vi "Read Device - Protocol.vi"(8 "error in (no error)":errorcluster, 11 "LTE in":refnum<class "LTE.lvclass">) -> (0 "error out":errorcluster, 2 "Device - Protocol":T1, 3 "LTE out":refnum<class "LTE.lvclass">)   [LabVIEW 2023, in "ANRITSU Call Box.lvlib" / "LTE.lvclass"]
uses:
  LTE.lvclass
  LTE.lvclass/LTE.ctl
  Type Definition/Call Device - Protocol Type Selector.ctl
  ANRITSU Call Box.lvlib
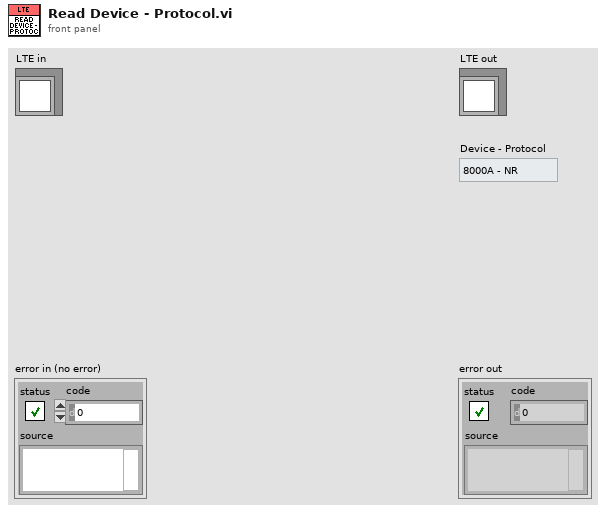
[diagram p1: front panel]
types:
  T1 = typedef "ANRITSU Call Box.lvlib/Call Device - Protocol Type Selector.ctl" = enum16{"8000A - NR", "8000A - LTE", "882xC - LTE"}
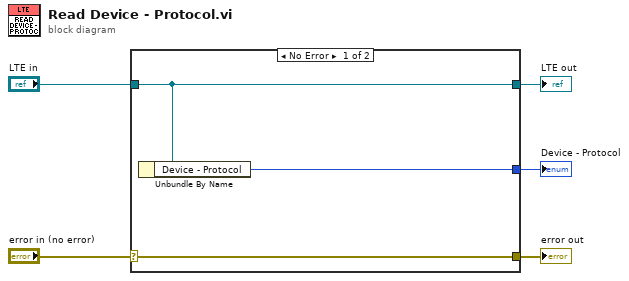
[diagram p0: block diagram]
diagram:
  n1 = case shown="No Error" "error in (no error)" {
    selector: "error in (no error)" -> [w8 w9]
    tunnel: [w8 w9] -> w4
    tunnel: [w7 w10] -> w2
    tunnel: "LTE in" -> [w7 w10]
    tunnel: [w6 _] -> w1
    frame No Error {
      n2 = Unbundle By Name(w7) -> ("Device - Protocol"=w6:T1)
    }
    frame Error {
    }
  }
  "error out" <- w4
  "LTE out" <- w2
  "Device - Protocol" <- w1
